vi "demo.vi"() -> ()   [LabVIEW 2020]
panel:
  out "percent complete":u32
  out "error out":errorcluster
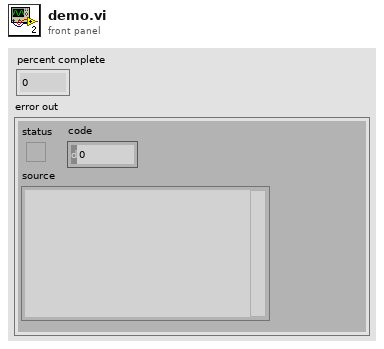
[diagram p1: front panel]
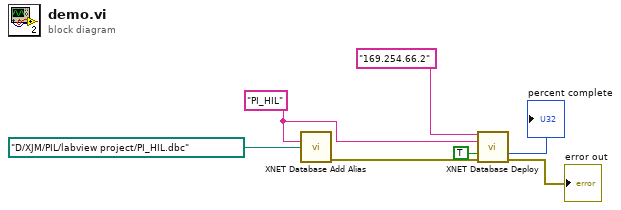
[diagram p0: block diagram]
diagram:
  w4 = "PI_HIL" ("alias")
  n1 = call <vilib>:"XNET Database Add Alias.vi"("alias"=w4, "filepath"=path "D:/XJM/PIL/labview project/PI_HIL.dbc") -> ("error out"=w6:errorcluster)  [unwired: 13 in]
  n2 = call <vilib>:"XNET Database Deploy.vi"("IP address"="169.254.66.2", "alias"=w4, "wait for complete? (true)"=TRUE, "error in (no error)"=w6) -> ("percent complete"=→"percent complete":u32, "error out"=→"error out":errorcluster)  [unwired: 10 in]
